vi "recycle_omit.vi"(11 "1folder names":string[](array[string])) -> (3 "Array":string[](array[string]))   [LabVIEW 2018]
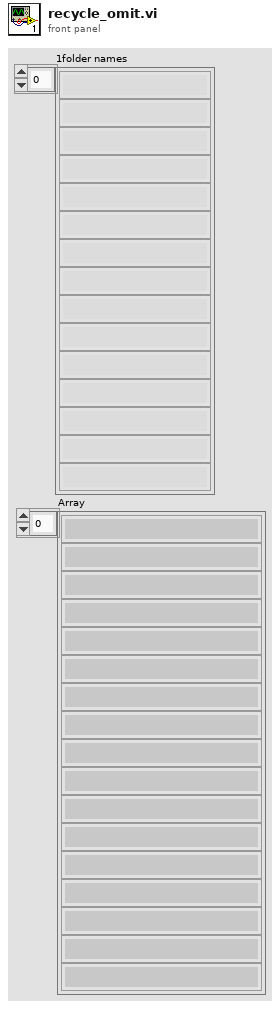
[diagram p1: front panel]
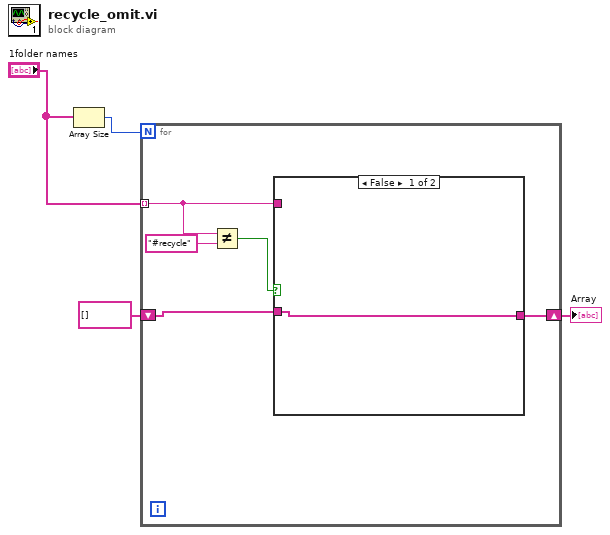
[diagram p0: block diagram]
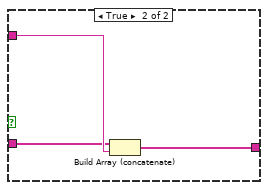
[diagram p2: hidden frame]
diagram:
  n1 = Array Size(array="1folder names") -> (size(s)=w4:i32)
  n2 = for {
    N: w4 -> [_]
    tunnel: "1folder names" -> [w7] mode=indexing
    shift-right: [w6] -> w1
    shift-left: string[] [] -> [w5]
    n3 = Not Equal?(x=w7, y="#recycle") -> (x != y?=w8:bool)
    n4 = case shown="False" w8 {
      tunnel: w7 -> [_ w13]
      tunnel: [w10 w12] -> w6
      tunnel: w5 -> [w10 w11]
      frame False {
      }
      frame True {
        n5 = Build Array (concatenate)(w11, w13) -> (w12:string[])
      }
    }
  }
  "Array" <- w1
